vi "Test Get-Set Data Name.vi"(8 "error in (no error)":errorcluster, 10 "types to test":variant[](array[variant])) -> (0 "error out":errorcluster, 2 "Passed":bool)   [LabVIEW 2020, in "test_openg_array.lvlib"]
uses:
  test_openg_array.lvlib
  <vilib>/addons/_JKI Toolkits/Caraya/classes/Test/Test.lvclass
  <vilib>/Utility/Data Type/NI_Data Type.lvlib
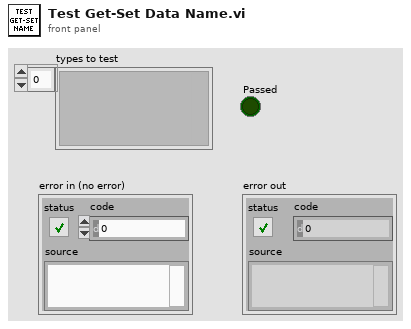
[diagram p1: front panel]
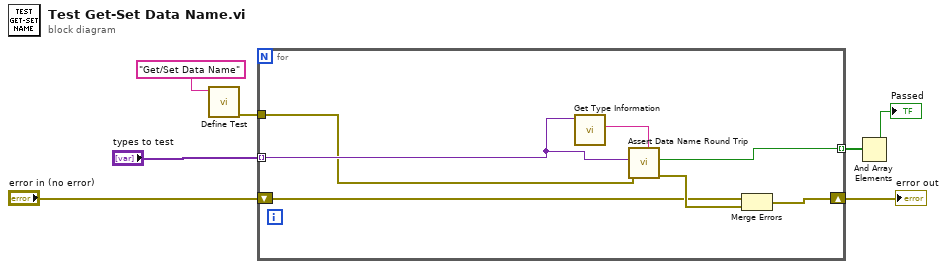
[diagram p0: block diagram]
diagram:
  n1 = call <vilib>:"Define Test.vi"("Label (VI Title)"="Get/Set Data Name") -> ("error out"=w7:errorcluster)  [unwired: 9 in, 1 out]
  n2 = for {
    tunnel: "types to test" -> [w13] mode=indexing
    shift-right: [w10] -> w2
    shift-left: "error in (no error)" -> [w9]
    tunnel: [w8] -> w4 mode=indexing
    tunnel: w7 -> [w12]
    n3 = call <vilib>:"Get Type Information.vi"("variant"=w13) -> ("name"=w14:string)  [unwired: 6 in, 4 out]
    n4 = call "Assert Data Name Round Trip.vi"("Label"=w14, "error in (no error)"=w12, "Variant"=w13) -> ("error out"=w11:errorcluster, "pass"=w8:bool)  [unwired: 7 in]
    n5 = Merge Errors(w9, w11) -> (w10:errorcluster)
  }
  "error out" <- w2
  n6 = And Array Elements(Boolean array=w4) -> (logical AND=→"Passed":bool)
